vi "Go.vi"(6 "Route":string, 8 "error in (no error)":errorcluster, 11 "Navigator in":refnum<class "Navigator.lvclass">) -> (0 "error out":errorcluster, 3 "Navigator out":refnum<class "Navigator.lvclass">)   [LabVIEW 2024, in "Navigator.lvclass"]
doc: "Clear Navigator stack and push route."
uses:
  Navigator.lvclass
  Navigator.lvclass/Navigator.ctl
  NavigatableView/NavigatableView.lvclass
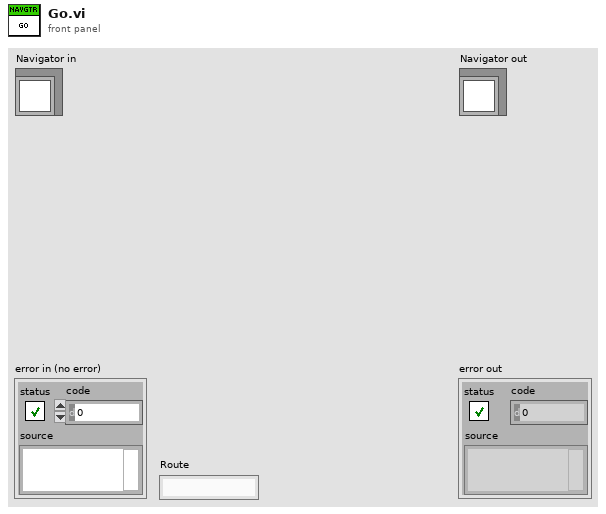
[diagram p1: front panel]
types:
  T1 = typedef "Navigator.lvclass/Route.ctl" = cluster{"Name":string, "Path":path, "Builder":refnum<class "NavigatableView.lvclass">}
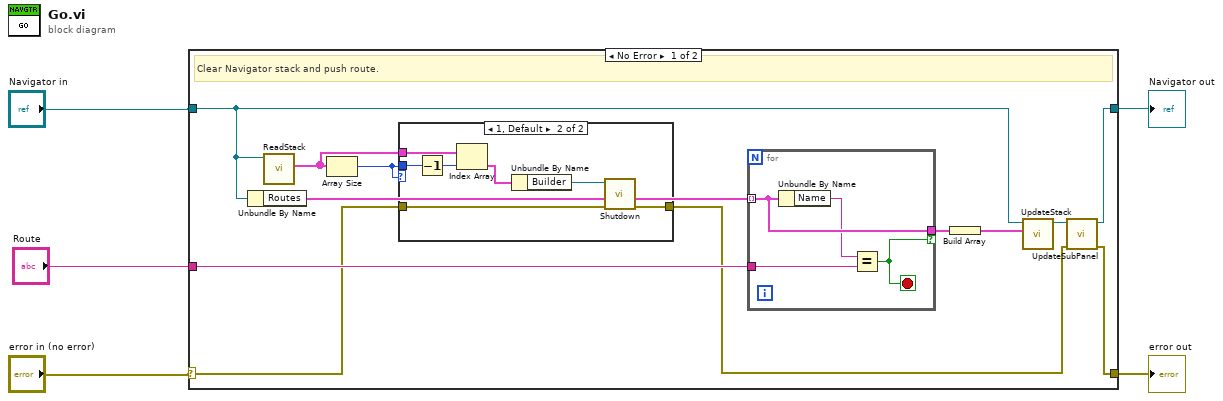
[diagram p0: block diagram]
diagram:
  n1 = case shown="No Error" "error in (no error)" {
    selector: "error in (no error)" -> [w14 w31]
    tunnel: [w11 w31] -> w4
    tunnel: [w12 w30] -> w5
    tunnel: "Navigator in" -> [w9 w30]
    tunnel: "Route" -> [w16 _]
    frame No Error {
      # "Clear Navigator stack and push route."
      n2 = Unbundle By Name(w9) -> ("Routes"=w17:T1[])
      n3 = call "ReadStack.vi"("Navigator in"=w9) -> ("Stack"=w7:T1[])  [unwired: 8 in, 2 out]
      n4 = Array Size(array=w7) -> (size(s)=w6:i32)
      n5 = case shown="1, Default" w6 {
        tunnel: w14 -> [w18 w25]
        tunnel: [w18 w24] -> w13
        tunnel: w6 -> [_ w22]
        tunnel: w7 -> [_ w20]
        frame 0 {
        }
        frame 1, Default {
          n6 = Decrement(x=w22) -> (x-1=w21:i32)
          n7 = Index Array(array=w20, index=w21) -> (element=w19:T1)
          n8 = Unbundle By Name(w19) -> ("Builder"=w23:refnum<class "NavigatableView.lvclass">)
          n9 = call-dynamic "Shutdown.vi"("error in (no error)"=w25, "NavigatableView in"=w23) -> ("error out"=w24:errorcluster)  [unwired: 8 in, 1 out]
        }
      }
      n10 = for {
        tunnel: w17 -> [w29] mode=indexing
        tunnel: [w29] -> w15 if=w26
        tunnel: w16 -> [w27]
        stop <- w26 stop-if-true
        n11 = Unbundle By Name(w29) -> ("Name"=w28:string)
        n12 = Equal?(x=w28, y=w27) -> (x = y?=w26:bool)
      }
      n13 = Build Array(w15) -> (w10:T1[])
      n14 = call "UpdateStack.vi"("Stack"=w10, "Navigator in"=w9) -> ("Navigator out"=w8:refnum<class "Navigator.lvclass">)  [unwired: 8 in, 1 out]
      n15 = call "UpdateSubPanel.vi"("error in (no error)"=w13, "Navigator in"=w8) -> ("error out"=w11:errorcluster, "Navigator out"=w12:refnum<class "Navigator.lvclass">)  [unwired: 8 in]
    }
    frame Error {
    }
  }
  "error out" <- w4
  "Navigator out" <- w5
